vi "UI Updater.vi"(10 "timeout [ms](30)":i32=30, 11 "update period [ms](15)":i32=15) -> ()   [LabVIEW 2018, in "GLog.lvlib" / "UI Updater.lvlib"]
uses:
  UI Updater.lvlib
  Handler Registration.ctl
  Indicator Data.ctl
  Events/Register.ctl
  6e2b1530-34a9-4714-a609-5ea4836b5261.vi
  b00cbca9-bfcb-4288-853c-af1aaf9f8f24.vi
panel:
  out "errors":errorcluster[](array[cluster])
  # "Connector Pane"
  # "Locals"
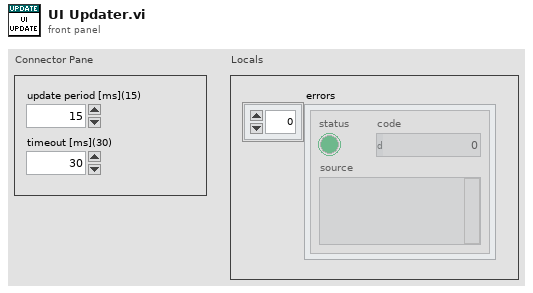
[diagram p1: front panel]
types:
  T1 = typedef "GLog.lvlib/UI Updater.lvlib/Indicator Data.ctl" = cluster{"Ctl Ref":refnum<vi>, "Log Buffer":string[], "Log Limit":i32, "Line Limit":i32, "Autoscroll?":bool, "Valid?":bool, "Owning VI":refnum<vi>, "Ctl Index":i32, "Needs Write?":bool}
  T2 = typedef "GLog.lvlib/UI Updater.lvlib/Handler Registration.ctl" = cluster{"handler name":string, "index":i32}
  T3 = typedef "GLog.lvlib/UI Updater.lvlib/Events.ctl" = cluster{"Write Log":refnum<user-event>, "Register":refnum<user-event>, "Unregister":refnum<user-event>}
  T4 = typedef "GLog.lvlib/UI Updater.lvlib/Register.ctl" = cluster{"Handler Name":string, "Ctl Ref":refnum<vi>, "Log Limit":i32, "Line Limit":i32, "AutoScroll?":bool}
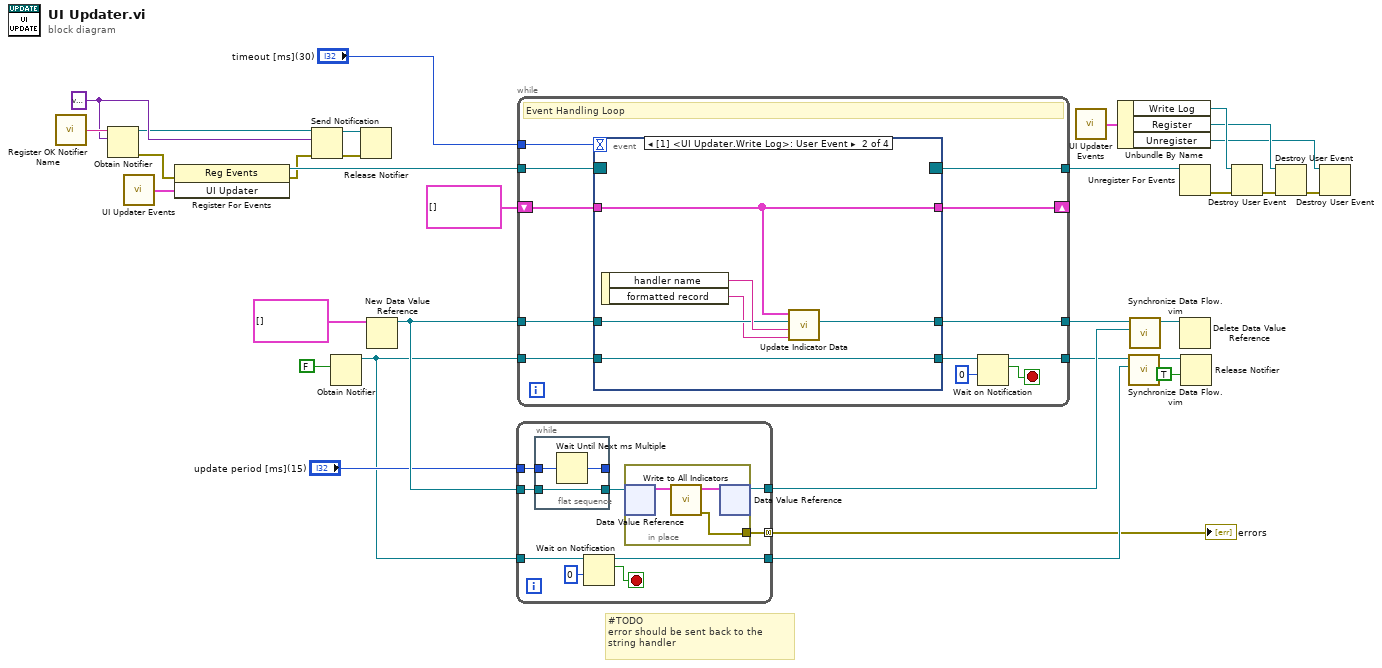
[diagram p0: block diagram]
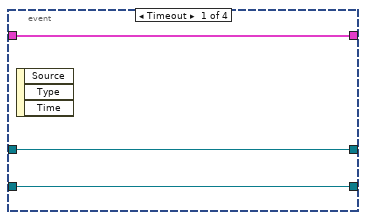
[diagram p2: hidden frame]
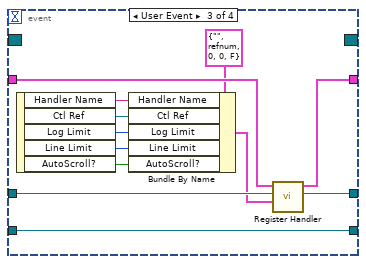
[diagram p3: hidden frame]
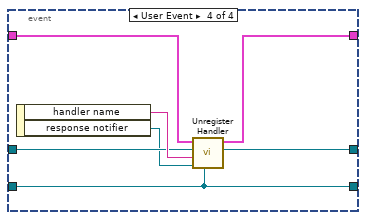
[diagram p4: hidden frame]
diagram:
  w12 = variant
  # "#TODO\nerror should be sent back to the string handler"
  n1 = call "Register OK Notifier Name.vi"() -> ("register ok notifier"=w13:string)  [unwired: 1 in]
  n2 = Obtain Notifier(name (unnamed)=w13, notification data type=w12) -> (notifier out=w11:refnum<notifier>, error out=w10:errorcluster)  [unwired: 2 in, 1 out]
  n3 = call "UI Updater Events.vi"() -> ("UI Updater"=w16:T3)  [unwired: 1 in]
  n4 = register-events(error in=w10, w16) -> (reference out=w25:refnum<event-registration>, error out=w9:errorcluster)  [unwired: 1 in]
  n5 = Send Notification(notification=w12, notifier=w11, error in (no error)=w9) -> (notifier out=w15:refnum<notifier>, error out=w14:errorcluster)
  n6 = Obtain Notifier(notification data type=FALSE) -> (notifier out=w28:refnum<notifier>)  [unwired: 3 in, 2 out]
  n7 = Release Notifier(notifier=w15, error in (no error)=w14) -> ()  [unwired: 1 in, 3 out]
  n8 = New Data Value Reference(data value=T1[] []) -> (data value reference=w32:refnum<data-value>)  [unwired: 1 in, 1 out]
  n9 = while {
    tunnel: "update period [ms](15)" -> [w40]
    tunnel: w28 -> [w36]
    tunnel: [w34] -> w21
    tunnel: w32 -> [w38]
    tunnel: [w41] -> w23
    tunnel: [w33] -> w8 mode=concatenating
    stop <- w37 stop-if-true
    n10 = flat-sequence {
      tunnel: w40 -> [w44]
      tunnel: [w43] -> w39
      tunnel: w38 -> [w43]
      tunnel: [w42] -> _
      frame #0 {
        n11 = Wait Until Next ms Multiple(millisecond multiple=w44) -> (millisecond timer value=w42:u32)
      }
    }
    n12 = Wait on Notification(notifier=w36, timeout in ms (-1)=0) -> (notifier out=w34:refnum<notifier>, notification=w37:bool)  [unwired: 2 in, 2 out]
    n13 = in-place {
      in-place-border: [w45] -> w33
      n14 = in-place-dvr #1(w39) -> (w47:T1[])  [unwired: 1 out]
      n15 = call "Write to All Indicators.vi"("indicator data in"=w47) -> ("errors"=w45:errorcluster[], "indicator data out"=w46:T1[])  [unwired: 9 in]
      n16 = in-place-dvr #1(w46) -> (w41:refnum<data-value>)  [unwired: 1 out]
    }
  }
  "errors" <- w8
  n17 = while {
    shift-right: [w54] -> _
    shift-left: T2[] [] ("Array") -> [w57]
    tunnel: "timeout [ms](30)" -> [w48]
    tunnel: w28 -> [w53]
    tunnel: [w51] -> w20
    tunnel: w32 -> [w58]
    tunnel: [w56] -> w24
    tunnel: w25 -> [w59]
    tunnel: [w55] -> w26
    stop <- w50 stop-if-true
    # "Event Handling Loop"
    n18 = event shown="[1] <UI Updater.Write Log>: User Event" {
      selector: w59 -> [_ _ _ _]
      dyn-events: [_ _ _ _] -> w55
      timeout: w48 -> [_ _ _ _]
      tunnel: w58 -> [w62 w66 w79 w85]
      tunnel: w57 -> [w61 w65 w78 w87]
      tunnel: [w62 w63 w77 w84] -> w56
      tunnel: [w61 w65 w76 w83] -> w54
      tunnel: w53 -> [w60 w67 w80 w81]
      tunnel: [w60 w67 w80 w81] -> w52
      event Timeout {
        n19 = event-data() -> ()  [unwired: 1 in, 3 out]
      }
      event User Event {
        n20 = event-data() -> ("handler name"=w68:string, "formatted record"=w64:string)  [unwired: 1 in]
        n21 = call "Update Indicator Data.vi"("formatted record"=w64, "handler name"=w68, "indicator data in"=w66, "registry in"=w65) -> ("indicator data out"=w63:refnum<data-value>)  [unwired: 7 in]
      }
      event User Event {
        n22 = event-data() -> ("Handler Name"=w74:string, "Ctl Ref"=w73:refnum<vi>, "Log Limit"=w72:i32, "Line Limit"=w71:i32, "AutoScroll?"=w70:bool)  [unwired: 1 in]
        n23 = Bundle By Name(cluster=T4 {"Handler Name"="", "Ctl Ref"=refnum, "Log Limit"=0, "Line Limit"=0, "AutoScroll?"=FALSE} ("Register"), "Handler Name"=w74, "Ctl Ref"=w73, "Log Limit"=w72, "Line Limit"=w71, "AutoScroll?"=w70) -> (w69:T4)
        n24 = call "Register Handler.vi"("registration data"=w69, "indicator data in"=w79, "registry in"=w78) -> ("indicator data out"=w77:refnum<data-value>, "registry out"=w76:T2[])  [unwired: 7 in]
      }
      event User Event {
        n25 = event-data() -> ("handler name"=w86:string, "response notifier"=w82:refnum<notifier>)  [unwired: 1 in]
        n26 = call "Unregister Handler.vi"("stop notifier"=w81, "response notifier"=w82, "handler name"=w86, "indicator data in"=w85, "registry in"=w87) -> ("indicator data out"=w84:refnum<data-value>, "registry out"=w83:T2[])  [unwired: 5 in]
      }
    }
    n27 = Wait on Notification(notifier=w52, timeout in ms (-1)=0) -> (notifier out=w51:refnum<notifier>, notification=w50:bool)  [unwired: 2 in, 2 out]
  }
  n28 = call "UI Updater Events.vi"() -> ("UI Updater"=w7:T3)  [unwired: 1 in]
  n29 = Unbundle By Name(w7) -> ("Write Log"=w6:refnum<user-event>, "Register"=w5:refnum<user-event>, "Unregister"=w4:refnum<user-event>)
  n30 = call "Synchronize Data Flow.vim"("input 2"=w21, "input 1"=w20) -> ("output 1"=w19:refnum<notifier>)  [unwired: 2 in, 3 out]
  n31 = call "Synchronize Data Flow.vim"("input 2"=w23, "input 1"=w24) -> ("output 1"=w22:refnum<data-value>)  [unwired: 2 in, 3 out]
  n32 = Unregister For Events(event registration refnum=w26) -> (error out=w3:errorcluster)  [unwired: 1 in]
  n33 = Delete Data Value Reference(data value reference=w22) -> ()  [unwired: 1 in, 2 out]
  n34 = Release Notifier(notifier=w19, force destroy? (F)=TRUE) -> ()  [unwired: 1 in, 3 out]
  n35 = Destroy User Event(user event=w6, error in=w3) -> (error out=w2:errorcluster)
  n36 = Destroy User Event(user event=w5, error in=w2) -> (error out=w1:errorcluster)
  n37 = Destroy User Event(user event=w4, error in=w1) -> ()  [unwired: 1 out]
